vi "Publish.vi"(4 "timeout (1000ms)":i32=1000, 5 "RETAIN":bool, 6 "QoS":T1, 7 "DUP (Re-delivery attempt)":bool, 8 "error in (no error)":errorcluster, 9 "Payload":variant, 10 "Topic Name (empty: Payload name)":string, 11 "Client in":refnum<class "Client.lvclass">) -> (0 "error out":errorcluster, 2 "Published":bool, 3 "Client out":refnum<class "Client.lvclass">)   [LabVIEW 2013, in "MQTT Client.lvlib" / "Client.lvclass"]
uses:
  Client.lvclass
  <vilib>/LabVIEW Open Source Project/MQTT Control Packets/Control Packets/ControlPacket/QualityOfService -- enum.ctl
  <vilib>/LabVIEW Open Source Project/MQTT Connection/MQTT_Base/Base Class/MQTT_Base.lvclass/MQTT_Base.ctl
  <vilib>/LabVIEW Open Source Project/Data Manipulation/TypeDescriptor/TypeDescriptor_GetName.vi
  <vilib>/LabVIEW Open Source Project/Data Manipulation/TypeDescriptor/TypeDescriptor_GetPString.vi
  <vilib>/LabVIEW Open Source Project/MQTT Connection/MQTT_Base/Base Class/MQTT_Base.lvclass
  <vilib>/LabVIEW Open Source Project/Data Manipulation/Variant/OpenVariant.lvlib
  <vilib>/LabVIEW Open Source Project/OpenSerializer/Serializer/Serializer.lvclass
  <vilib>/LabVIEW Open Source Project/MQTT Control Packets/Control Packets/ControlPacket/ControlPacket.lvclass
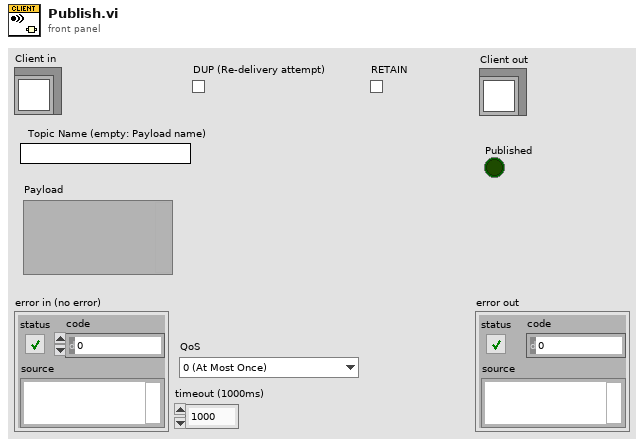
[diagram p1: front panel]
types:
  T1 = typedef "MQTT_Control_Packets.lvlib/ControlPacket.lvclass/QualityOfService -- enum.ctl" = enum16{"0 (At Most Once)", "1 (At Least Once)", "2 (Exactly Once)"}
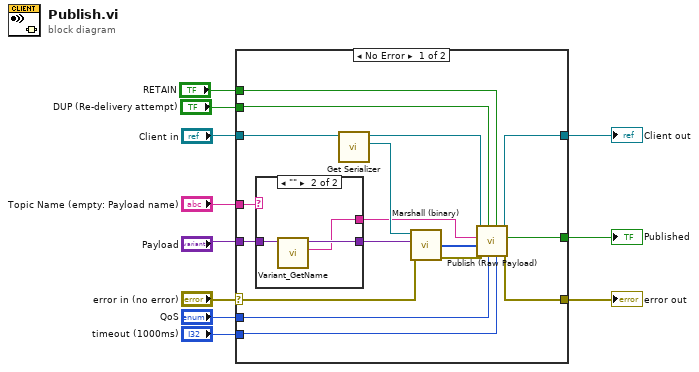
[diagram p0: block diagram]
diagram:
  n1 = case shown="No Error" "error in (no error)" {
    selector: "error in (no error)" -> [w24 w35]
    tunnel: [w13 w35] -> w6
    tunnel: [w20 w34] -> w7
    tunnel: "Client in" -> [w25 w34]
    tunnel: "Payload" -> [w28 _]
    tunnel: "Topic Name (empty: Payload name)" -> [w27 _]
    tunnel: "QoS" -> [w17 _]
    tunnel: "timeout (1000ms)" -> [w18 _]
    tunnel: [w26 _] -> w3
    tunnel: "DUP (Re-delivery attempt)" -> [w16 _]
    tunnel: "RETAIN" -> [w12 _]
    frame No Error {
      n2 = case shown="\"\"" w27 {
        selector: w27 -> [w30 _]
        tunnel: w28 -> [w29 w33]
        tunnel: [w29 w32] -> w23
        tunnel: [w30 w31] -> w15
        frame Default {
        }
        frame "" {
          n3 = call <vilib>:"Variant_GetName.vi"("Variant"=w33) -> ("Name"=w31:string, "Variant dup"=w32:variant)  [unwired: 8 in, 1 out]
        }
      }
      n4 = call <vilib>:"Get Serializer.vi"("MQTT_Base"=w25) -> ("Serializer"=w22:refnum<class "Serializer.lvclass">, "MQTT_Base out"=w19:refnum<class "Client.lvclass">)  [unwired: 8 in, 1 out]
      n5 = call <vilib>:"Marshall (binary).vi"("error in (no error)"=w24, "Variant"=w23, "Serializer in"=w22) -> ("error out"=w21:errorcluster, "Bytes"=w14:u8[])  [unwired: 6 in, 1 out]
      n6 = call "Publish (Raw Payload).vi"("timeout (1000ms)"=w18, "RETAIN"=w12, "QoS"=w17, "DUP (Re-delivery attempt)"=w16, "error in (no error)"=w21, "Binary Payload"=w14, "Topic Name"=w15, "Client in"=w19) -> ("error out"=w13:errorcluster, "Published"=w26:bool, "Client out"=w20:refnum<class "Client.lvclass">)  [unwired: 1 in]
    }
    frame Error {
    }
  }
  "error out" <- w6
  "Client out" <- w7
  "Published" <- w3
